vi "PicoScope4000aGetAnalogueOffset.vi"(8 "error in (no error)":errorcluster, 9 "Coupling":u32(ring) items=["AC", "DC"], 10 "Range":u32(ring) items=["10mV", "20mV", "50mV", "100mV", "200mV", "500mV", "1V", "2V", "5V", "10V", "20V", "50V", "100V", "200V", "1KV_2_5V", "1KV_5V", "1KV_12_5V", "1KV_25V", "1KV_50V", "1KV_125V", "1KV_250V", "1KV_500V", "1KV_1000V", "CURRENT_CLAMP_200A_2kA_1A", "CURRENT_CLAMP_200A_2kA_2A", "CURRENT_CLAMP_200A_2kA_5A", "CURRENT_CLAMP_200A_2kA_10A", "CURRENT_CLAMP_200A_2kA_20A", "CURRENT_CLAMP_200A_2kA_50A", "CURRENT_CLAMP_200A_2kA_100A", "CURRENT_CLAMP_200A_2kA_200A", "CURRENT_CLAMP_200A_2kA_500A", "CURRENT_CLAMP_200A_2kA_1000A", "CURRENT_CLAMP_200A_2kA_2000A", "CURRENT_CLAMP_40A_100mA", "CURRENT_CLAMP_40A_200mA", "CURRENT_CLAMP_40A_500mA", "CURRENT_CLAMP_40A_1A", "CURRENT_CLAMP_40A_2A", "CURRENT_CLAMP_40A_5A", "CURRENT_CLAMP_40A_10A", "CURRENT_CLAMP_40A_20A", "CURRENT_CLAMP_40A_40A", "CURRENT_CLAMP_2000ARMS_10A", "CURRENT_CLAMP_2000ARMS_20A", "CURRENT_CLAMP_2000ARMS_50A", "CURRENT_CLAMP_2000ARMS_100A", "CURRENT_CLAMP_2000ARMS_200A", "CURRENT_CLAMP_2000ARMS_500A", "CURRENT_CLAMP_2000ARMS_1000A", "CURRENT_CLAMP_2000ARMS_2000A", "CURRENT_CLAMP_2000ARMS_5000A", "x10_Probe_100mV", "x10_Probe_200mV", "x10_Probe_500mV", "x10_Probe_1V", "x10_Probe_2V", "x10_Probe_5V", "x10_Probe_10V", "x10_Probe_20V", "x10_Probe_50V", "x10_Probe_100V", "x10_Probe_200V", "x10_Probe_500V", "CURRENT_CLAMP_60A_2A", "CURRENT_CLAMP_60A_5A", "CURRENT_CLAMP_60A_10A", "CURRENT_CLAMP_60A_20A", "CURRENT_CLAMP_60A_50A", "CURRENT_CLAMP_60A_60A", "CURRENT_CLAMP_60A_V2_0_5A", "CURRENT_CLAMP_60A_V2_1A", "CURRENT_CLAMP_60A_V2_2A", "CURRENT_CLAMP_60A_V2_5A", "CURRENT_CLAMP_60A_V2_10A", "CURRENT_CLAMP_60A_V2_20A", "CURRENT_CLAMP_60A_V2_50A", "CURRENT_CLAMP_60A_V2_60A", "RESISTANCE_LEAD_NEG5_TO_20OHM", "RESISTANCE_LEAD_NEG50_TO_200OHM", "RESISTANCE_LEAD_NEG500_TO_2KOHM", "RESISTANCE_LEAD_NEG5K_TO_20KOHM", "RESISTANCE_LEAD_NEG50K_TO_LEAD_200KOHM", "RESISTANCE_LEAD_NEG500K_TO_LEAD_2MOHM", "RESISTANCE_LEAD_DIODE_TEST", "HT_NEG3_TO_5KV", "HT_NEG3_TO_10KV", "HT_NEG5_TO_20KV", "HT_NEG5_TO_50KV", "HT_NEG5_TO_100KV", "HT_NEG3_TO_5KV_INVERTED", "HT_NEG3_TO_10KV_INVERTED", "HT_NEG5_TO_20KV_INVERTED", "HT_NEG5_TO_50KV_INVERTED", "HT_NEG5_TO_100KV_INVERTED", "TEMPERATURE_NEG50_TO_150DEGC", "PRESSURE_SENSOR_-100k-150k_PASCALS", "PRESSURE_SENSOR_-100k_TO_400k_PASCALS", "PRESSURE_SENSOR_-200k_TO_800k_PASCALS", "PRESSURE_SENSOR_-400k_TO_1600k_PASCALS", "PRESSURE_SENSOR_-400k_TO_3400k_PASCALS", "PRESSURE_SENSOR_-150k_TO_1350k_PASCALS"], 11 "handle in":i16) -> (0 "error out":errorcluster, 1 "minimumValue":sgl, 2 "maximumValue":sgl, 3 "handle out":i16)   [LabVIEW 2009]
doc: "Calls GetAnalogueOffset"
uses:
  Program Files/Pico Technology/SDK/lib/ps4000a.dll
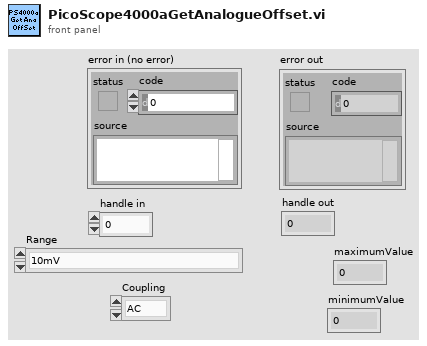
[diagram p1: front panel]
types:
  T1 = cluster{"status":bool, "code":u32, "source":string}
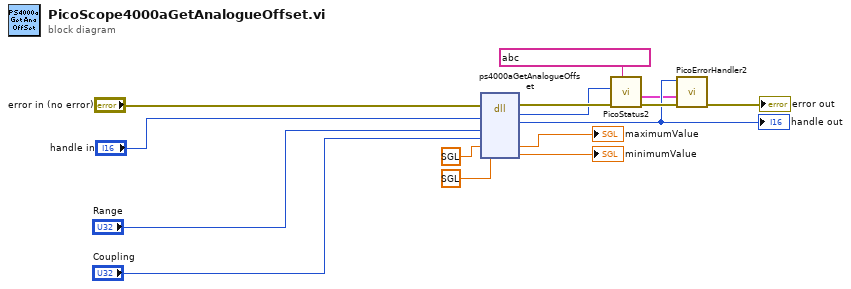
[diagram p0: block diagram]
diagram:
  n1 = dll-call lib="/Program Files/Pico Technology/SDK/lib/ps4000a.dll" fn="ps4000aGetAnalogueOffset" ("ps3000.dll:_ps3000_open_unit@0")(error in="error in (no error)", "handle"="handle in", "range"="Range", "coupling"="Coupling", "maximumVoltage"=sgl ?, "minimumVoltage"=sgl ?) -> (error out=w6:errorcluster, "PICO_STATUS"=w4:u32, "handle"=w3:i16, "maximumVoltage"=→"maximumValue":sgl, "minimumVoltage"=→"minimumValue":sgl)  [unwired: 4 in, 1 out]
  "handle out" <- w3
  n2 = call "PicoStatus2.vi"("PICO source"=string ? ("source"), "Error in"=w6, "PICO STATUS"=w4) -> ("error out"=w7:errorcluster, "PICO_STATUS out"=w1:T1)  [unwired: 5 in]
  n3 = call "PicoErrorHandler2.vi"("error in (no error)"=w7, "PICO_STATUS in"=w1, "handle In"=w3) -> ("error out"=→"error out":errorcluster)  [unwired: 8 in]
